vi "Test First Enqueued Return Value is Returned when Recording Expectation.vi"(8 "error in (no error)":errorcluster, 11 "Test Case In":refnum<class "Return Value Test.lvclass">) -> (0 "error out":errorcluster, 3 "Test Case Out":refnum<class "Return Value Test.lvclass">)   [LabVIEW 2020, in "Return Value Test.lvclass"]
uses:
  Return Value Test.lvclass
  C:/Program Files (x86)/National Instruments/LabVIEW 2020/vi.lib/Astemes/LUnit/Test Case.lvclass
  <vilib>/Astemes/LUnit/Test Case.lvclass/Test Case.ctl
  4993e8ee-a06a-463a-9684-69129f64d5ce.vi
  Test Doubles/Test Interface Responsive Mock/Test Interface Mock.lvclass
  source/Expectations/One/One.lvlib
  <vilib>/Astemes/LUnit/Test Case.lvclass
  C:/git/astemes-lmock/source/Framework/Mock/Mock.lvclass
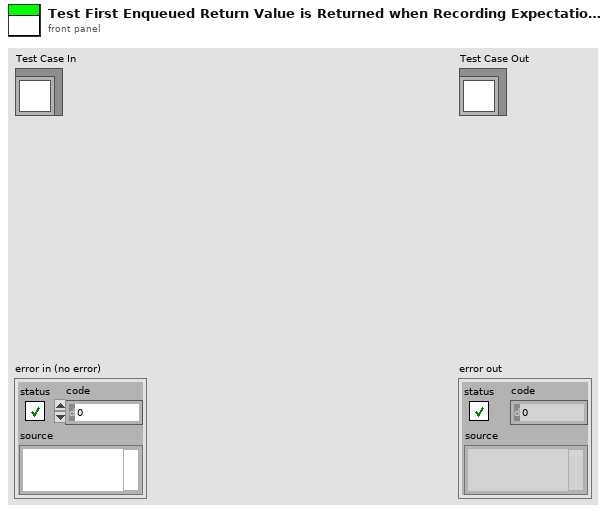
[diagram p1: front panel]
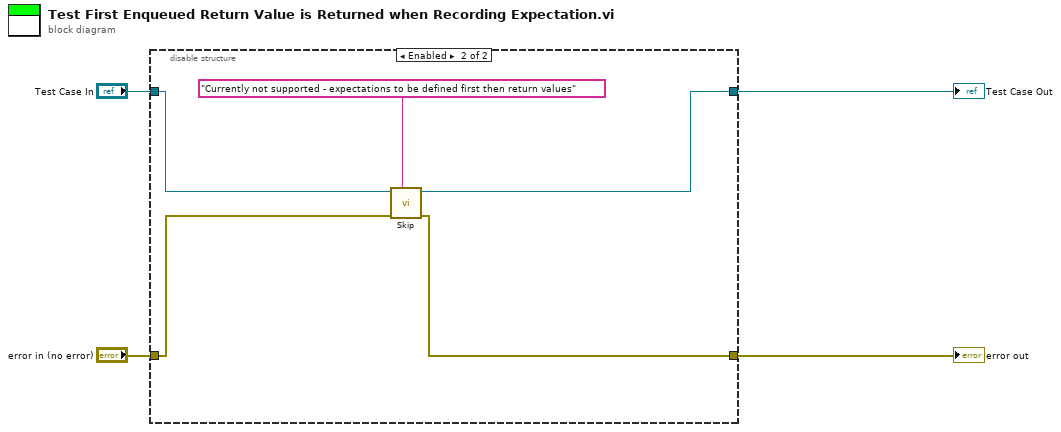
[diagram p0: block diagram]
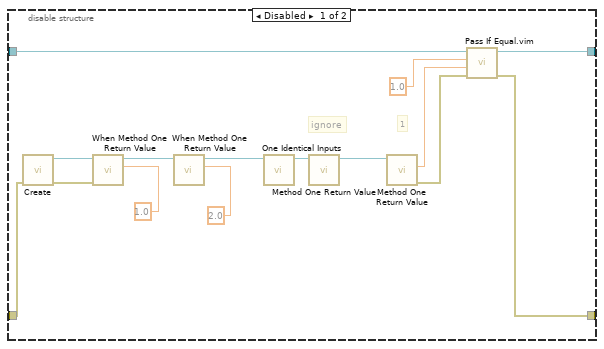
[diagram p2: hidden frame]
diagram:
  n1 = disable-structure shown="Enabled" {
    disable-tunnel: "Test Case In" -> [w19 w23]
    disable-tunnel: "error in (no error)" -> [w14 w24]
    disable-tunnel: [w5 w22] -> w2
    disable-tunnel: [w6 w21] -> w1
    frame Disabled {
      # "ignore"
      # "1"
      n2 = call "Create.vi"("error in (no error)"=w14) -> ("error out"=w17:errorcluster, "Test Interface Mock Out"=w18:refnum<class "Test Interface Mock.lvclass">)  [unwired: 9 in]
      n3 = call "When Method One Return Value.vi"("Return Value"=1.0, "error in (no error)"=w17, "Test Interface Mock In"=w18) -> ("Test Interface Mock Out"=w16:refnum<class "Test Interface Mock.lvclass">)  [unwired: 8 in]
      n4 = call "When Method One Return Value.vi"("Return Value"=2.0, "Test Interface Mock In"=w16) -> ("Test Interface Mock Out"=w13:refnum<class "Test Interface Mock.lvclass">)  [unwired: 9 in]
      n5 = call "One Identical Inputs.vi"("Mock in"=w13) -> ("Mock out"=w8:refnum<class "Test Interface Mock.lvclass">)  [unwired: 9 in, 1 out]
      n6 = call-dynamic "Method One Return Value.vi"("Test Interface Mock in"=w8) -> ("Test Interface Mock out"=w7:refnum<class "Test Interface Mock.lvclass">)  [unwired: 8 in, 2 out]
      n7 = call-dynamic "Method One Return Value.vi"("Test Interface Mock in"=w7) -> ("error out"=w15:errorcluster, "Return Value"=w9:dbl)  [unwired: 8 in, 1 out]
      n8 = call "Pass If Equal.vim"("error in (no error)"=w15, "Actual"=w9, "Expected"=1.0 ("Return Value"), "LUnit Test Case In"=w19) -> ("error out"=w5:errorcluster, "LUnit Test Case Out"=w6:refnum<class "Return Value Test.lvclass">)  [unwired: 6 in]
    }
    frame Enabled {
      n9 = call <vilib>:"Skip.vi"("Description"="Currently not supported - expectations to be defined first then return values", "error in (no error)"=w24, "LUnit Test Case In"=w23) -> ("error out"=w22:errorcluster, "LUnit Test Case Out"=w21:refnum<class "Return Value Test.lvclass">)  [unwired: 7 in]
    }
  }
  "error out" <- w2
  "Test Case Out" <- w1
